vi "example_cmd.vi"() -> ()   [LabVIEW 2021]
doc: "This examples launches the cmd.exe process and allows you to send strings via stdin, while asynchronously listening to stdout and stderr \n\nCalling \"exit\" in CmdIn will stop the cmd.exe instance and stop this VI. You can leverage this by adding a final exit line after the command(s)\nyou wish to send to have this VI auto-terminate upon completion."
uses:
  dotnet_system_exec/dotnet_system_exec.lvclass
panel:
  out "ExitCode":i32
  in  "working directory":path=path "c:/"
  out "StdErr":string
  out "StdOut":string
  in  "Send":bool
  in  "Cmd In (can include multiple lines)":string="dir"
  in  "Stop":bool
  # "This examples launches the cmd.exe process and allows you to send strings via stdin, while asynchronously listening to stdout and stderr  \n\nCalling \"exit\" in CmdIn will stop the cmd.exe instance and stop this VI. You can leverage this by adding a final exit line after the command(s)\nyou wish to send to have this VI auto-terminate upon completion."
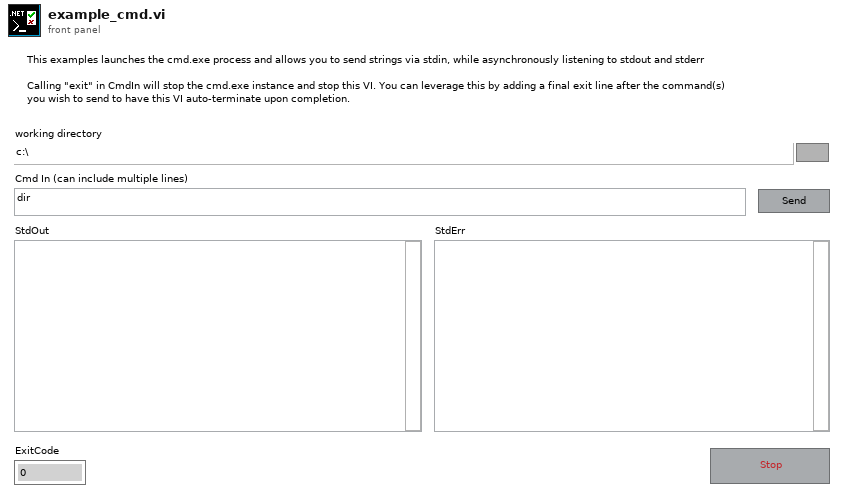
[diagram p1: front panel]
types:
  T1 = cluster{"StdOut Event":refnum<user-event>, "StdErr Event":refnum<user-event>, "ProcessExit Event":refnum<user-event>}
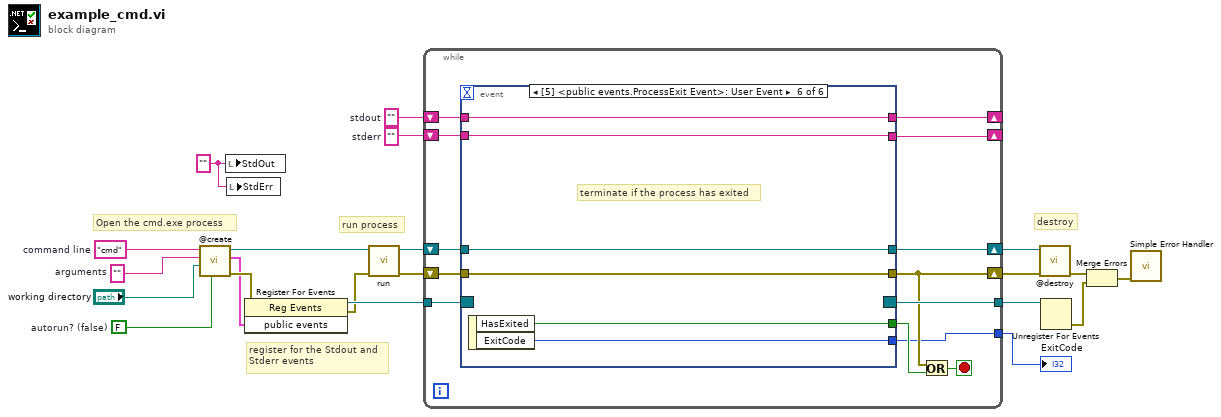
[diagram p0: block diagram]
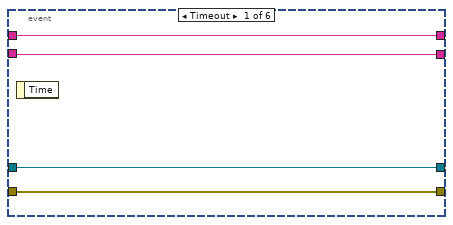
[diagram p2: hidden frame]
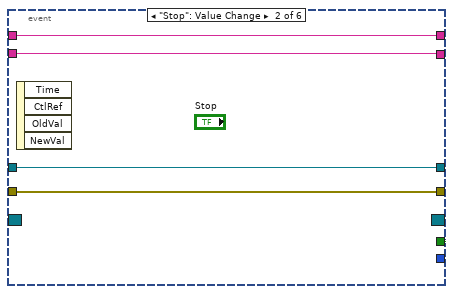
[diagram p3: hidden frame]
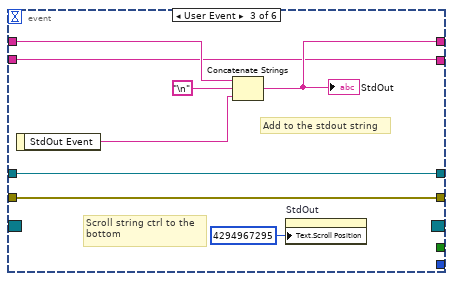
[diagram p4: hidden frame]
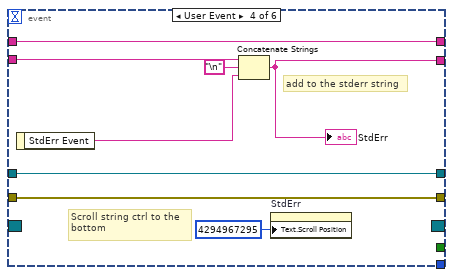
[diagram p5: hidden frame]
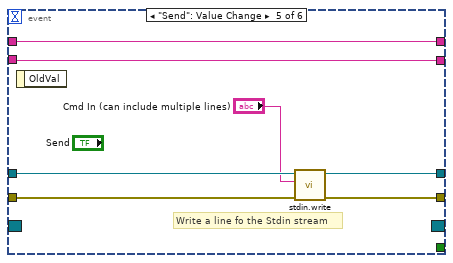
[diagram p6: hidden frame]
diagram:
  w2 = FALSE  # autorun? (false)
  w3 = "" ("Process File Name")
  w5 = ""  # stderr
  w10 = ""  # arguments
  w11 = ""  # stdout
  w12 = "cmd"  # command line
  # "destroy"
  # "register for the Stdout and\nStderr events"
  # "run process"
  # "Open the cmd.exe process"
  n1 = call "@create.vi"("autorun? (false)"=w2, "working directory (c:\\)"="working directory", "arguments (\"\")"=w10, "command line (cmd.exe)"=w12) -> ("error out"=w8:errorcluster, "public events"=w6:T1, "dotnet_system_exec out"=w19:refnum<class "dotnet_system_exec.lvclass">)  [unwired: 5 in]
  n2 = local write "StdOut"(w3) -> ()
  n3 = local write "StdErr"(w3) -> ()
  n4 = register-events(error in=w8, w6) -> (reference out=w18:refnum<event-registration>, error out=w7:errorcluster)  [unwired: 1 in]
  n5 = call "run.vi"("error in (no error)"=w7, "dotnet_system_exec in"=w19) -> ("error out"=w9:errorcluster, "dotnet_system_exec out"=w21:refnum<class "dotnet_system_exec.lvclass">)  [unwired: 8 in]
  n6 = while {
    shift-right: [w34] -> w20
    shift-left: w21 -> [w33]
    shift-right: [w24] -> w16
    shift-left: w9 -> [w32]
    tunnel: w18 -> [w31]
    tunnel: [w30] -> w17
    shift-right: [w28] -> _
    shift-left: w11 -> [w29]
    shift-right: [w26] -> _
    shift-left: w5 -> [w27]
    tunnel: [w22] -> w1
    stop <- w23 stop-if-true
    n7 = event shown="[5] <public events.ProcessExit Event>: User Event" {
      selector: w31 -> [_ _ _ _ _ _]
      dyn-events: [_ _ _ _ _ _] -> w30
      timeout: _ -> [_ _ _ _ _ _]
      tunnel: [w38 w43 w51 w59 w66 w69] -> w34
      tunnel: w33 -> [w38 w43 w51 w59 w65 w69]
      tunnel: w32 -> [w37 w42 w50 w58 w63 w68]
      tunnel: [w37 w42 w50 w58 w64 w68] -> w24
      tunnel: w29 -> [w36 w40 w47 w54 w61 w70]
      tunnel: [w36 w40 w48 w54 w61 w70] -> w28
      tunnel: [_ TRUE _ _ _ w72] -> w25
      tunnel: w27 -> [w35 w39 w45 w55 w60 w71]
      tunnel: [w35 w39 w45 w53 w60 w71] -> w26
      tunnel: [_ _ _ _ _ w67] -> w22
      event Timeout {
        n8 = event-data() -> ()  [unwired: 1 in, 1 out]
      }
      event "Stop": Value Change {
        n9 = event-data() -> ()  [unwired: 1 in, 4 out]
      }
      event User Event {
        # "Scroll string ctrl to the \nbottom"
        # "Add to the stdout string"
        n10 = event-data() -> ("StdOut Event"=w46:string)  [unwired: 1 in]
        n11 = Concatenate Strings(w47, "\n", w46) -> (w48:string)
        "StdOut" <- w48
        n12 = property on="StdOut" class="Str"("Text.Scroll Position"=u32 4294967295) -> ()  [unwired: 2 in, 2 out]
      }
      event User Event {
        # "Scroll string ctrl to the \nbottom"
        # "add to the stderr string"
        n13 = event-data() -> ("StdErr Event"=w56:string)  [unwired: 1 in]
        n14 = Concatenate Strings(w55, "\n", w56) -> (w53:string)
        "StdErr" <- w53
        n15 = property on="StdErr" class="Str"("Text.Scroll Position"=u32 4294967295) -> ()  [unwired: 2 in, 2 out]
      }
      event "Send": Value Change {
        # "Write a line fo the Stdin stream"
        n16 = event-data() -> ()  [unwired: 1 in, 1 out]
        n17 = call-dynamic "stdin.write.vi"("error in (no error)"=w63, "stdin"="Cmd In (can include multiple lines)", "dotnet_system_exec in"=w65) -> ("error out"=w64:errorcluster, "dotnet_system_exec out"=w66:refnum<class "dotnet_system_exec.lvclass">)  [unwired: 7 in]
      }
      event User Event {
        # "terminate if the process has exited"
        n18 = event-data() -> ("HasExited"=w72:bool, "ExitCode"=w67:i32)  [unwired: 1 in]
      }
    }
    n19 = Or(x=w24, y=w25) -> (x .or. y?=w23:bool)
  }
  "ExitCode" <- w1
  n20 = call-dynamic "@destroy.vi"("error in (no error)"=w16, "dotnet_system_exec in"=w20) -> ("error out"=w15:errorcluster)  [unwired: 8 in, 1 out]
  n21 = Unregister For Events(event registration refnum=w17) -> (error out=w14:errorcluster)  [unwired: 1 in]
  n22 = Merge Errors(w15, w14) -> (w13:errorcluster)
  n23 = call <vilib>:"Simple Error Handler.vi"("error in (no error)"=w13) -> ()  [unwired: 4 in, 5 out]
